vi "ReadConfiguration.vi"(8 "error in (no error)":errorcluster, 11 "object in":refnum<class "Channel.lvclass">) -> (0 "error out":errorcluster, 2 "Configuration":refnum<class "Configuration.lvclass">, 3 "object out":refnum<class "Channel.lvclass">)   [LabVIEW 2021, in "Channel.lvlib" / "Channel.lvclass"]
uses:
  Channel.lvclass
  Configuration_class/Configuration.lvclass
  Channel.lvclass/Channel.ctl
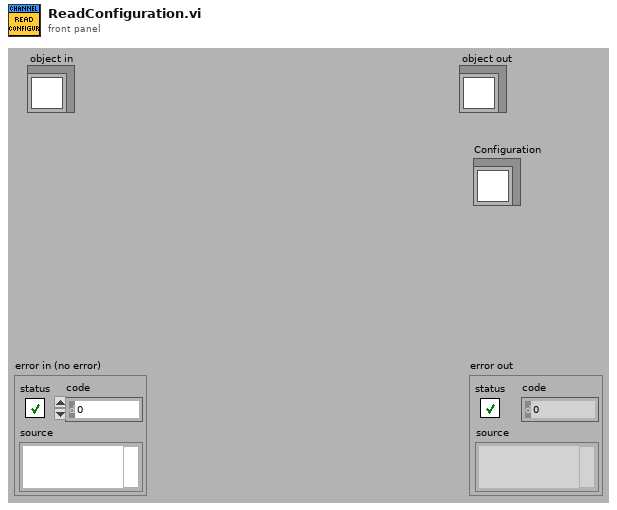
[diagram p1: front panel]
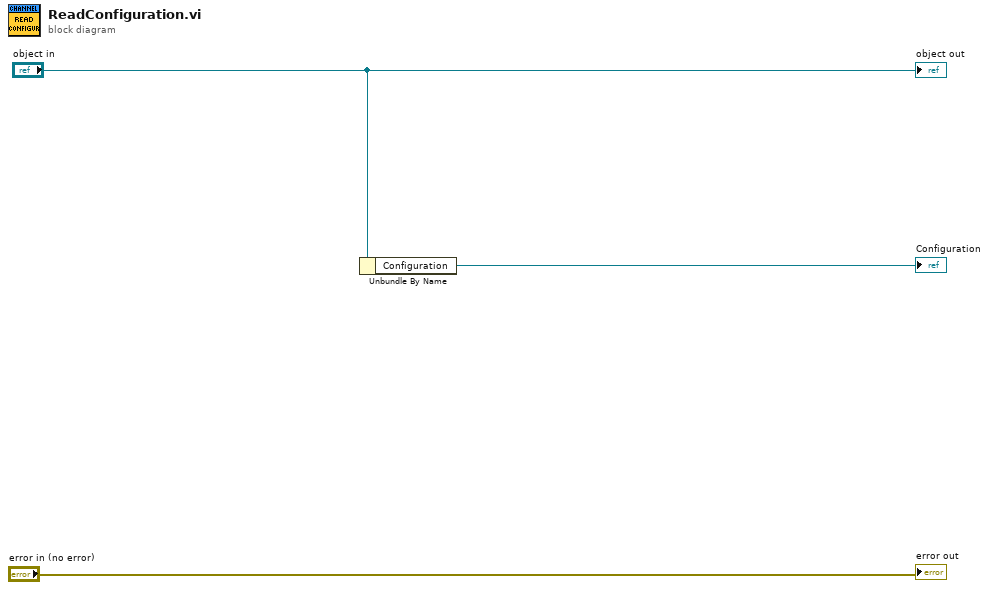
[diagram p0: block diagram]
diagram:
  n1 = Unbundle By Name("object in") -> ("Configuration"=→"Configuration":refnum<class "Configuration.lvclass">)
  "error out" <- "error in (no error)"
  "object out" <- "object in"
